vi "Sets and Query the Limit for the Compare Function.vi"(5 "Enable to Query":bool=TRUE, 7 "Enable to Sets":bool=TRUE, 8 "error in":errorcluster, 9 "Upper Limit Value":dbl=1.0 format="%.6e", 10 "Lower Limit Value":dbl format="%.6e", 11 "VISA resource name":refnum<visa-resource-name>) -> (0 "error out":errorcluster, 1 "Return the Upper Limit Value":string, 2 "Return the Lower Limit Value":string, 3 "VISA resource name out":refnum<visa-resource-name>)   [LabVIEW 2012, in "GDM-9052.lvlib"]
uses:
  GDM-9052.lvlib
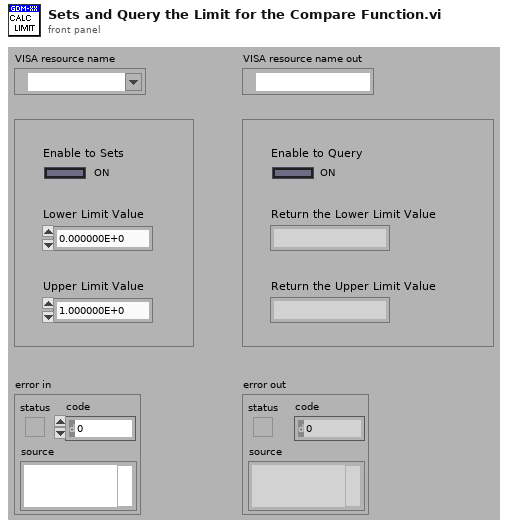
[diagram p1: front panel]
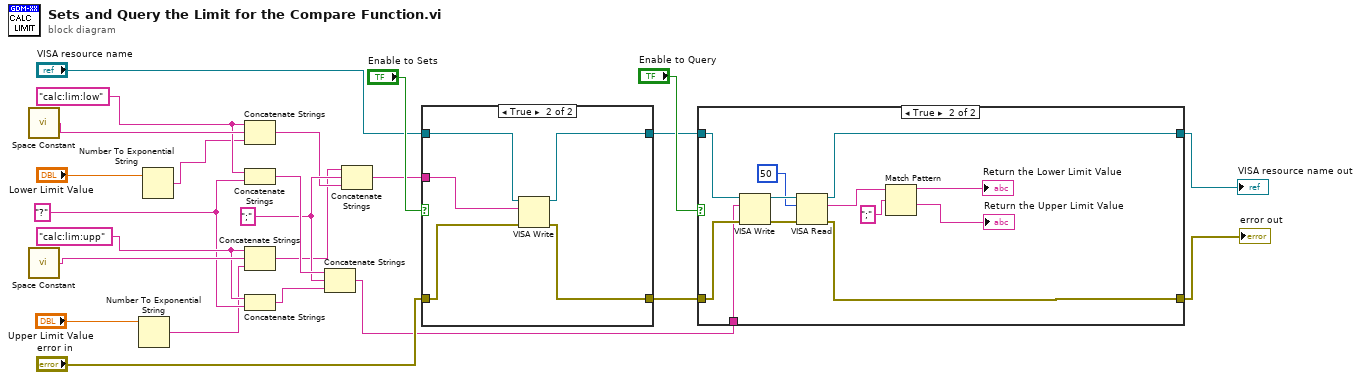
[diagram p0: block diagram]
diagram:
  w18 = ";" ("string")
  w20 = "?" ("string")
  w21 = "calc:lim:upp"
  w23 = "calc:lim:low"
  n1 = call <vilib>:"Space Constant.vi"() -> ("String"=w24:string)
  n2 = call <vilib>:"Space Constant.vi"() -> ("String"=w22:string)
  n3 = Number To Exponential String(number="Upper Limit Value") -> (E-format string=w3:string)  [unwired: 3 in]
  n4 = Number To Exponential String(number="Lower Limit Value") -> (E-format string=w5:string)  [unwired: 3 in]
  n5 = Concatenate Strings(w23, w24, w5) -> (w2:string)
  n6 = Concatenate Strings(w23, w20) -> (w19:string)
  n7 = Concatenate Strings(w21, w22, w3) -> (w1:string)
  n8 = Concatenate Strings(w21, w20) -> (w17:string)
  n9 = Concatenate Strings(w19, w18, w17) -> (w7:string)
  n10 = Concatenate Strings(w1, w18, w2) -> (w15:string)
  n11 = case shown="True" "Enable to Sets" {
    tunnel: w15 -> [_ w31]
    tunnel: "VISA resource name" -> [w26 w30]
    tunnel: "error in" -> [w25 w29]
    tunnel: [w26 w28] -> w11
    tunnel: [w25 w27] -> w10
    frame False {
    }
    frame True {
      n12 = VISA Write(VISA resource name=w30, write buffer=w31, error in (no error)=w29) -> (VISA resource name out=w28:refnum<visa-resource-name>, error out=w27:errorcluster)  [unwired: 1 out]
    }
  }
  n13 = case shown="True" "Enable to Query" {
    tunnel: w11 -> [w33 w42]
    tunnel: [w33 w39] -> w9
    tunnel: w10 -> [w32 w41]
    tunnel: [w32 w38] -> w8
    tunnel: w7 -> [_ w40]
    frame False {
    }
    frame True {
      n14 = VISA Write(VISA resource name=w42, write buffer=w40, error in (no error)=w41) -> (VISA resource name out=w44:refnum<visa-resource-name>, error out=w45:errorcluster)  [unwired: 1 out]
      n15 = VISA Read(VISA resource name=w44, byte count=u32 50, error in (no error)=w45) -> (VISA resource name out=w39:refnum<visa-resource-name>, read buffer=w37:string, error out=w38:errorcluster)  [unwired: 1 out]
      n16 = Match Pattern(string=w37, regular expression=";") -> (before substring=→"Return the Lower Limit Value":string, after substring=→"Return the Upper Limit Value":string)  [unwired: 1 in, 2 out]
    }
  }
  "VISA resource name out" <- w9
  "error out" <- w8
